vi "Check.vi"(9 "log line":string, 10 "current file":refnum<file>, 11 "size trigger in":refnum<class "RolloverTrigger.Size.lvclass">) -> (2 "rollover?":bool, 3 "size trigger out":refnum<class "RolloverTrigger.Size.lvclass">)   [LabVIEW 2018, in "GLog.lvlib" / "RolloverTrigger.Size.lvclass"]
doc: "Checks if the current file size exceeds the maximum file size."
uses:
  RolloverTrigger.Size.lvclass
  RolloverTrigger.Size.lvclass/RolloverTrigger.Size.ctl
  e9d6d0f3-f198-4e12-8664-206ea4c1767d.vi
panel:
  # "Connector Pane"
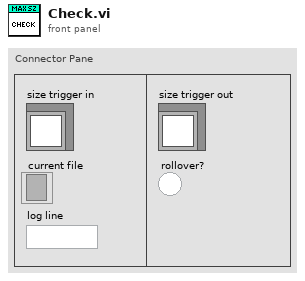
[diagram p1: front panel]
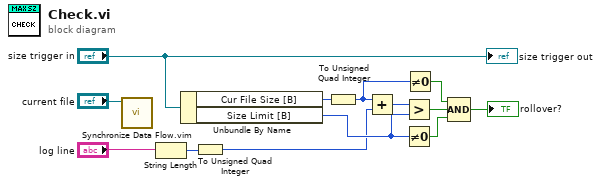
[diagram p0: block diagram]
diagram:
  n1 = call "Synchronize Data Flow.vim"("input 1"="current file") -> ()  [unwired: 3 in, 4 out]
  n2 = String Length(string="log line") -> (length=w6:i32)
  n3 = Unbundle By Name("size trigger in") -> ("Cur File Size [B]"=w12:i64, "Size Limit [B]"=w5:u64)
  n4 = To Unsigned Quad Integer(1:w6) -> (0:w4:u64)
  n5 = To Unsigned Quad Integer(1:w12) -> (0:w3:u64)
  n6 = Add(x=w3, y=w4) -> (x+y=w7:u64)
  n7 = Greater?(x=w7, y=w5) -> (0:w13:bool)
  n8 = Not Equal To 0?(x=w5) -> (x != 0?=w9:bool)
  n9 = Not Equal To 0?(x=w3) -> (x != 0?=w2:bool)
  n10 = Compound Arithmetic op=AND(w2, w13, w9) -> (→"rollover?":bool)
  "size trigger out" <- "size trigger in"
